vi "VIH HelpGen - HTML - Encode string to HTML format (strict).vi"(10 "Reject CR (T)":bool=TRUE, 11 "string":string) -> (3 "HTML string":string)   [LabVIEW 2014]
doc: "::: VI Helpeks :::\nCopyright (c) 2000-2026 Konstantin Shifershteyn. All rights reserved."
panel:
  # "VI Helpeks\nCopyright (c) 2012-2026 Konstantin Shifershteyn"
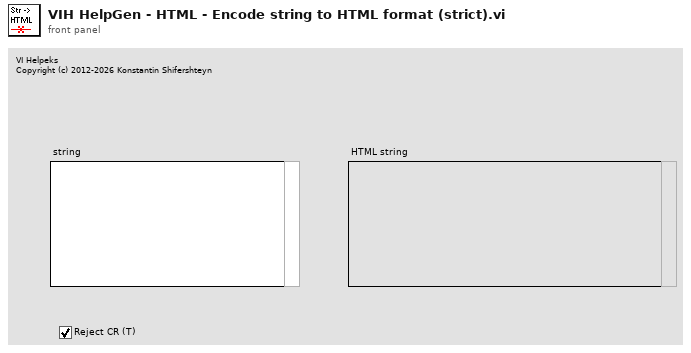
[diagram p1: front panel]
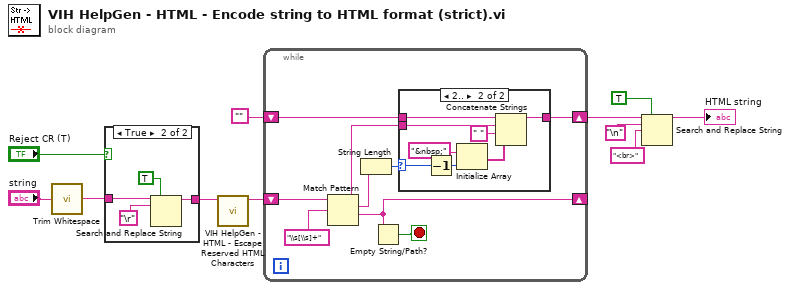
[diagram p0: block diagram]
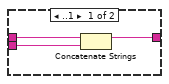
[diagram p2: hidden frame]
diagram:
  n1 = call <vilib>:"Trim Whitespace.vi"("string"="string") -> ("trimmed string"=w10:string)  [unwired: 1 in]
  n2 = case shown="True" "Reject CR (T)" {
    tunnel: w10 -> [w12 w16]
    tunnel: [w12 w15] -> w1
    frame False {
    }
    frame True {
      n3 = Search and Replace String(replace all?=TRUE, input string=w16, search string="\r") -> (result string=w15:string)  [unwired: 5 in, 3 out]
    }
  }
  n4 = call "VIH HelpGen - HTML - Escape Reserved HTML Characters.vi"("string"=w1) -> ("HTML string"=w3:string)  [unwired: 10 in]
  n5 = while {
    shift-right: [w23] -> _
    shift-left: w3 -> [w25]
    shift-right: [w20] -> w7
    shift-left: "" -> [w19]
    stop <- w22 stop-if-true
    n6 = Match Pattern(string=w25, regular expression="\\s[\\s]+") -> (before substring=w18:string, match substring=w21:string, after substring=w23:string)  [unwired: 1 in, 1 out]
    n7 = String Length(string=w21) -> (length=w17:i32)
    n8 = Empty String/Path?(string/path=w23) -> (empty?=w22:bool)
    n9 = case shown="2.." w17 {
      selector: w17 -> [_ w30]
      tunnel: [w26 w33] -> w20
      tunnel: w19 -> [w28 w32]
      tunnel: w18 -> [w27 w31]
      frame ..1 {
        n10 = Concatenate Strings(w28, w27) -> (w26:string)
      }
      frame 2.. {
        n11 = Decrement(x=w30) -> (x-1=w36:i32)
        n12 = Initialize Array("&nbsp;", w36) -> (w34:string[])
        n13 = Concatenate Strings(w32, w31, " " ("string"), w34) -> (w33:string)
      }
    }
  }
  n14 = Search and Replace String(replace all?=TRUE, input string=w7, search string="\n", replace string="<br>") -> (result string=→"HTML string":string)  [unwired: 4 in, 3 out]
